vi "BSD BR all info cluster.vi"(8 "R Table":string[][](table), 9 "R Table Tag":string[](array[string]), 10 "B Table Tag":string[](array[string]), 11 "B info":string[](array[string])) -> (3 "BR all info":T1)   [LabVIEW 2018]
panel:
  out "BR BL and STD info":T2
  out "B STD [pA]":dbl
  out "Region STD [pA]":dbl
  out "Region BL [pA]":dbl
  out "B BL [pA]":dbl
  out "BR info":T3
  out "Region STD [pA]":string
  out "Region BL [pA]":string
  out "B STD [pA]":string
  out "B BL [pA]":string
  out "R # [n]":string
  out "R info":string[](array[string])
  out "数値":i32
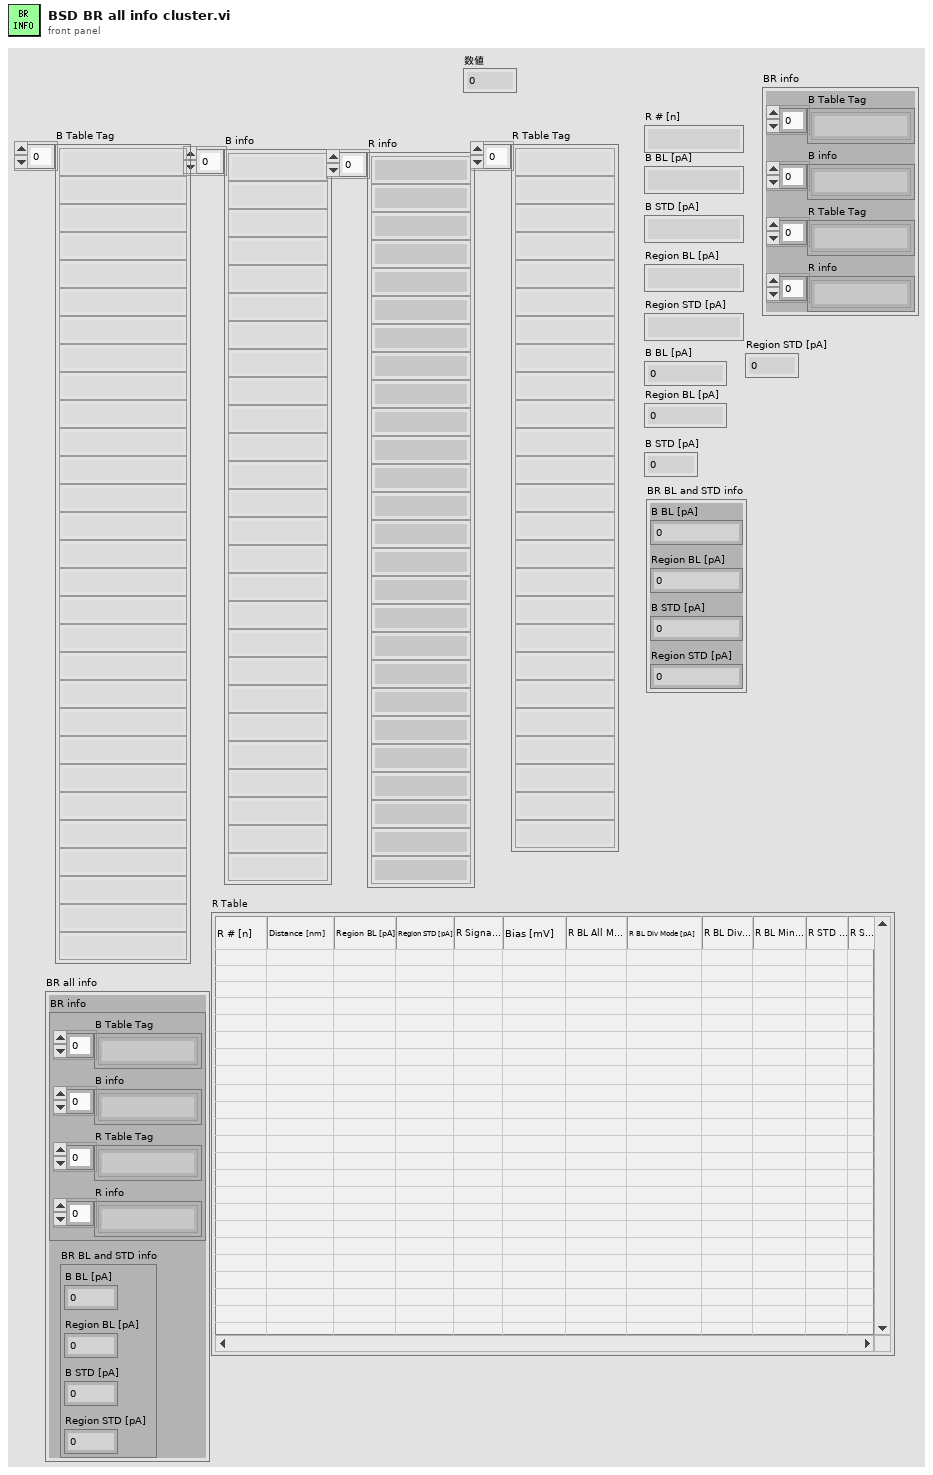
[diagram p1: front panel]
types:
  T1 = cluster{"BR info":cluster{"B Table Tag":string[], "B info":string[], "R Table Tag":string[], "R info":string[]}, "BR BL and STD info":cluster{"B BL [pA]":dbl, "Region BL [pA]":dbl, "B STD [pA]":dbl, "Region STD [pA]":dbl}}
  T2 = cluster{"B BL [pA]":dbl, "Region BL [pA]":dbl, "B STD [pA]":dbl, "Region STD [pA]":dbl}
  T3 = cluster{"B Table Tag":string[], "B info":string[], "R Table Tag":string[], "R info":string[]}
  T4 = cluster{"B Table Tag":string[], "B info":string[], "R Table Tag":string[], "R Table":string[]}
  T5 = cluster{cluster{"B Table Tag":string[], "B info":string[], "R Table Tag":string[], "R Table":string[]}, cluster{dbl, dbl, dbl, dbl}}
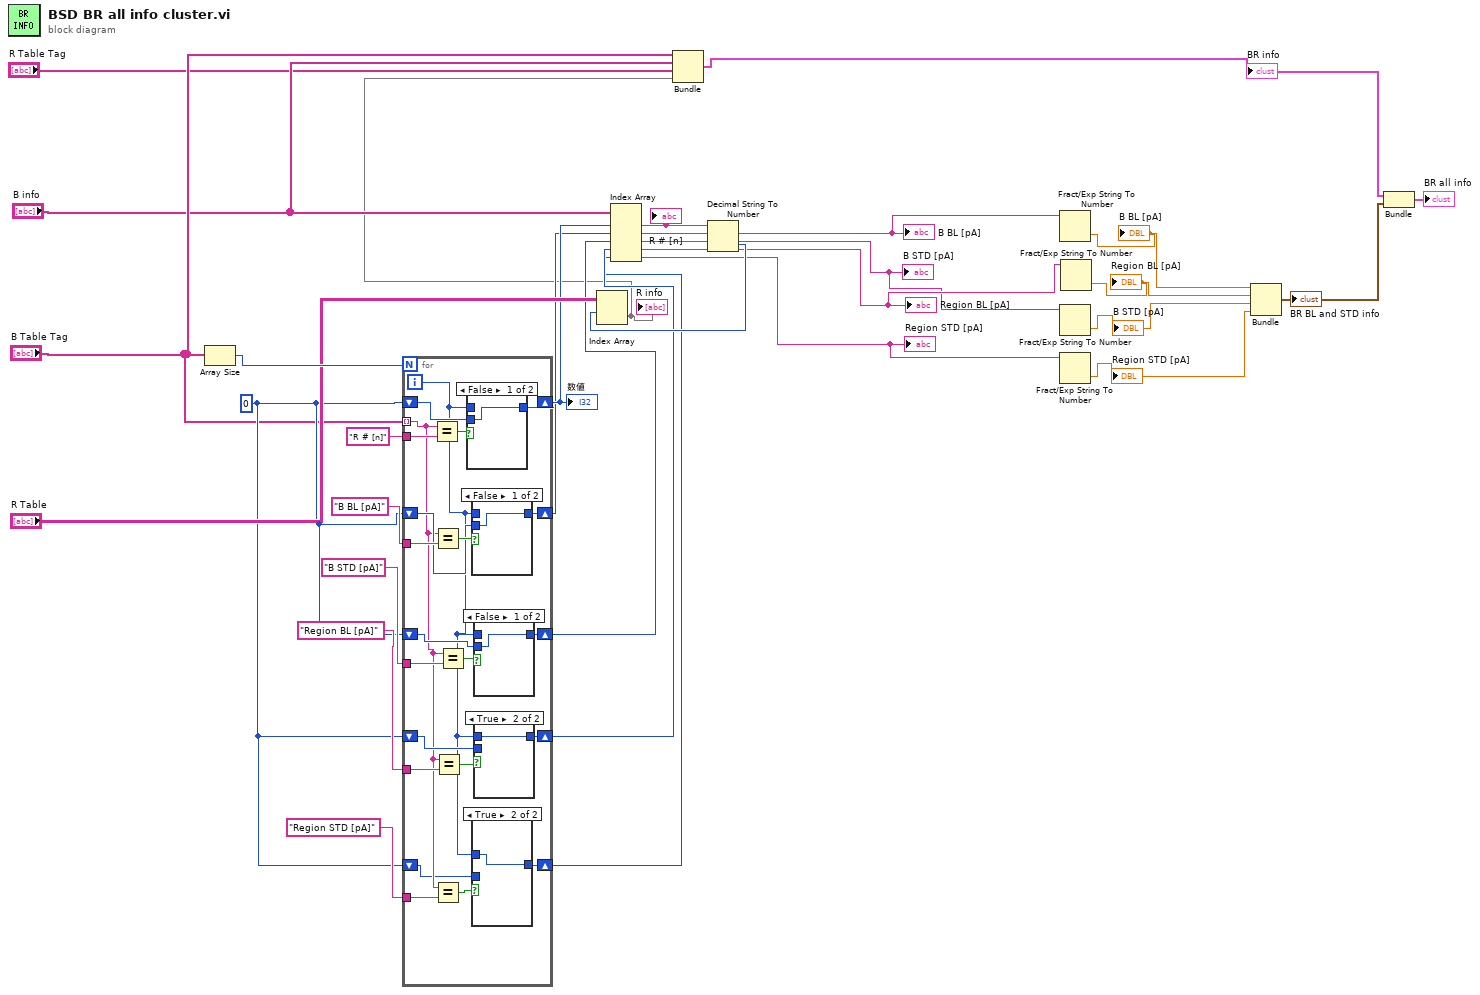
[diagram p0: block diagram]
diagram:
  w17 = 0
  n1 = Array Size(array="B Table Tag") -> (size(s)=w30:i32)
  n2 = for {
    N: w30 -> [_]
    tunnel: "B Table Tag" -> [w34] mode=indexing
    tunnel: "R # [n]" ("グループ名入力") -> [w52]
    shift-right: [w50] -> w27
    shift-left: w17 -> [w51]
    tunnel: "B BL [pA]" ("グループ名入力") -> [w45]
    tunnel: "B STD [pA]" ("グループ名入力") -> [w44]
    tunnel: "Region BL [pA]" ("グループ名入力") -> [w43]
    shift-right: [w42] -> w21
    shift-left: w17 -> [w39]
    shift-right: [w41] -> w20
    shift-left: w17 -> [w38]
    shift-right: [w40] -> w19
    shift-left: w17 -> [w37]
    tunnel: "Region STD [pA]" ("グループ名入力") -> [w36]
    shift-right: [w32] -> w16
    shift-left: w17 -> [w33]
    i -> [w31]
    n3 = Equal?(x=w34, y=w52) -> (x = y?=w49:bool)
    n4 = Equal?(x=w34, y=w45) -> (x = y?=w48:bool)
    n5 = Equal?(x=w34, y=w36) -> (x = y?=w35:bool)
    n6 = Equal?(x=w34, y=w43) -> (x = y?=w46:bool)
    n7 = Equal?(x=w34, y=w44) -> (x = y?=w47:bool)
    n8 = case shown="False" w49 {
      tunnel: w31 -> [_ w62]
      tunnel: [w61 w62] -> w50
      tunnel: w51 -> [w61 _]
      frame False {
      }
      frame True {
      }
    }
    n9 = case shown="False" w48 {
      tunnel: w31 -> [_ w60]
      tunnel: [w59 w60] -> w42
      tunnel: w39 -> [w59 _]
      frame False {
      }
      frame True {
      }
    }
    n10 = case shown="True" w35 {
      tunnel: [w53 w54] -> w32
      tunnel: w33 -> [w53 _]
      tunnel: w31 -> [_ w54]
      frame False {
      }
      frame True {
      }
    }
    n11 = case shown="False" w47 {
      tunnel: w31 -> [_ w58]
      tunnel: [w57 w58] -> w41
      tunnel: w38 -> [w57 _]
      frame False {
      }
      frame True {
      }
    }
    n12 = case shown="True" w46 {
      tunnel: w31 -> [_ w56]
      tunnel: [w55 w56] -> w40
      tunnel: w37 -> [w55 _]
      frame False {
      }
      frame True {
      }
    }
  }
  "数値" <- w27
  n13 = Index Array(array="B info", index #1=w27, index #2=w21, index #3=w20, index #4=w19, index #5=w16) -> (element #1=w26:string, element #2=w11:string, element #3=w9:string, element #4=w10:string, element #5=w8:string)
  "R # [n]" <- w26
  "B BL [pA]" <- w11
  "B STD [pA]" <- w9
  "Region BL [pA]" <- w10
  "Region STD [pA]" <- w8
  n14 = Decimal String To Number(string=w26) -> (number=w25:i32)  [unwired: 2 in, 1 out]
  n15 = Index Array(array="R Table", index (row)=w25) -> (element=w12:string[])  [unwired: 1 in]
  "R info" <- w12
  n16 = Bundle("B Table Tag"="B Table Tag", "B info"="B info", "R Table Tag"="R Table Tag", "R Table"=w12) -> (w2:T4)  [unwired: 1 in]
  "BR info" <- w2
  n17 = Fract/Exp String To Number(string=w11) -> (number=w7:dbl)  [unwired: 3 in, 1 out]
  "B BL [pA]" <- w7
  n18 = Fract/Exp String To Number(string=w9) -> (number=w5:dbl)  [unwired: 3 in, 1 out]
  "B STD [pA]" <- w5
  n19 = Fract/Exp String To Number(string=w8) -> (number=w4:dbl)  [unwired: 3 in, 1 out]
  "Region STD [pA]" <- w4
  n20 = Fract/Exp String To Number(string=w10) -> (number=w6:dbl)  [unwired: 3 in, 1 out]
  "Region BL [pA]" <- w6
  n21 = Bundle(w7, w6, w5, w4) -> (w1:cluster{dbl, dbl, dbl, dbl})  [unwired: 1 in]
  "BR BL and STD info" <- w1
  n22 = Bundle(w2, w1) -> (→"BR all info":T5)  [unwired: 1 in]
